vi "ContextManager.FGV.vi"(7 "context in":refnum<class "zmq_context.lvclass">, 10 "error in":errorcluster, 11 "action":T1) -> (2 "error out":errorcluster, 3 "context out":refnum<class "zmq_context.lvclass">, 5 "retired?":bool)   [LabVIEW 2019, in "RemoteControl.ZMQ.lvlib" / "ZMQ.ContextManager.lvlib"]
uses:
  ZMQ.ContextManager.lvlib
  <vilib>/addons/zeromq/zmq_context.lvclass
  Typedefs/Action--enum.ctl
  Typedefs/Context--Cluster.ctl
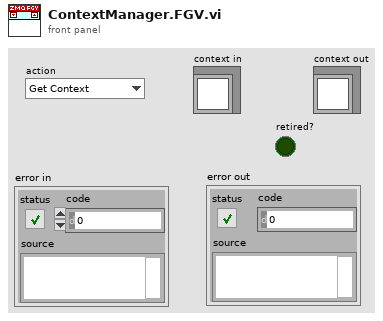
[diagram p1: front panel]
types:
  T1 = typedef "RemoteControl.ZMQ.lvlib/ZMQ.ContextManager.lvlib/Action--enum.ctl" = enum16{"Get Context", "Release Context", "Socket Opened", "Socket Closed", "Force Cleanup", "Set Context", "Retire If Idle"}
  T2 = typedef "RemoteControl.ZMQ.lvlib/ZMQ.ContextManager.lvlib/Context--Cluster.ctl" = cluster{"context":refnum<class "zmq_context.lvclass">, "context users":u32, "socket counter":u32, "idle since (ms)":u32}
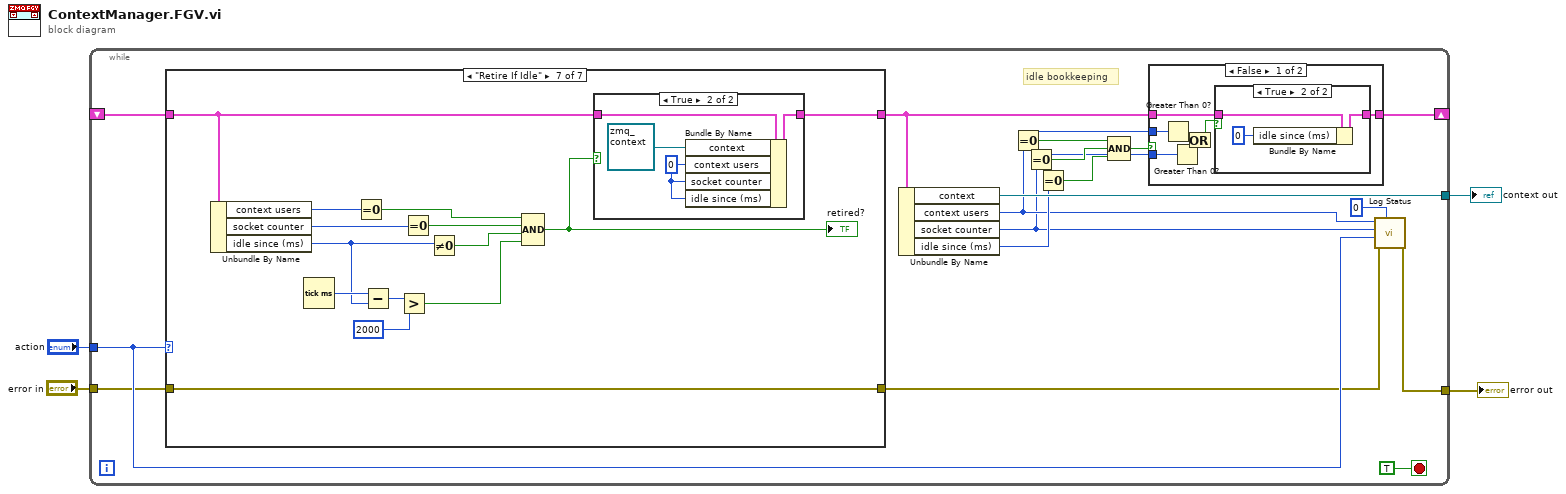
[diagram p0: block diagram]
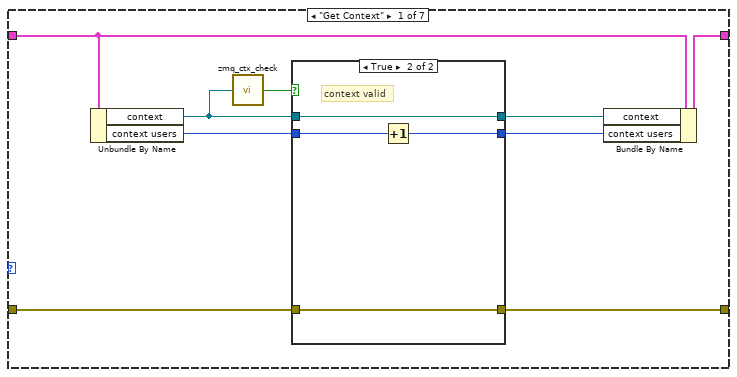
[diagram p2: hidden frame]
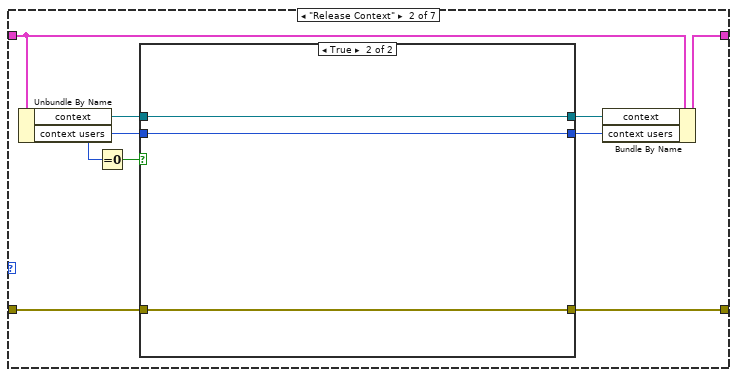
[diagram p4: hidden frame]
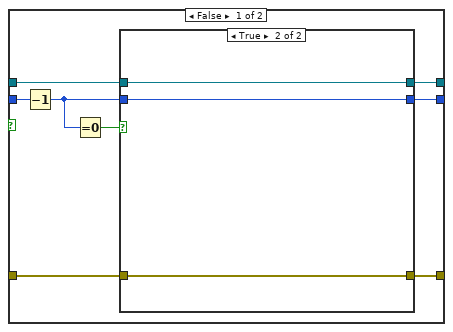
[diagram p5: hidden frame]
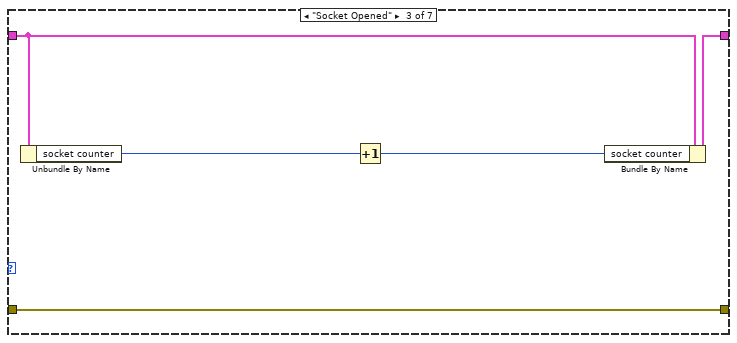
[diagram p7: hidden frame]
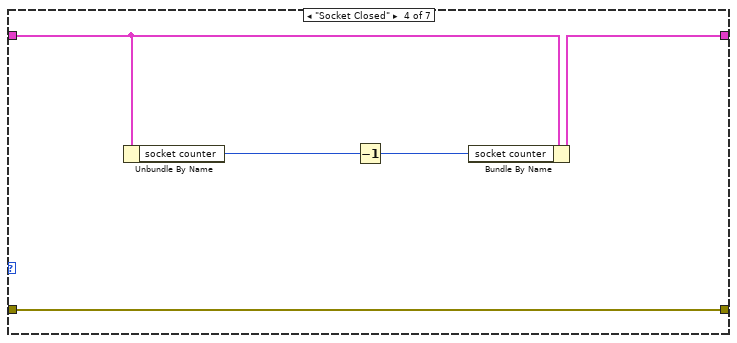
[diagram p8: hidden frame]
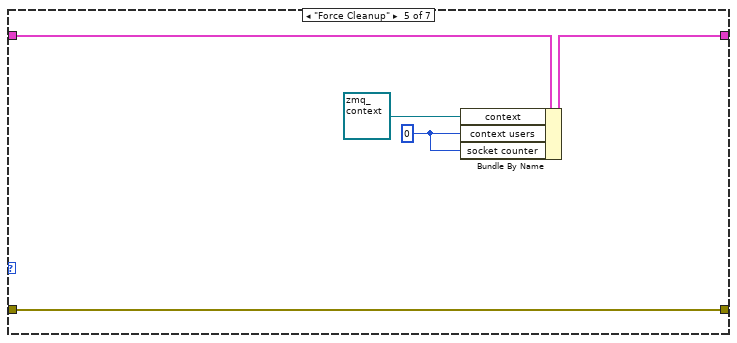
[diagram p9: hidden frame]
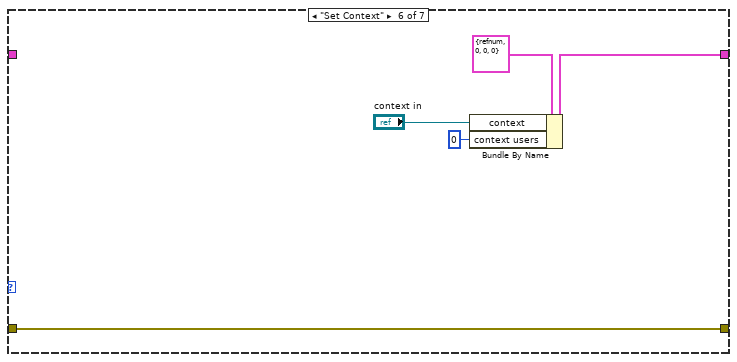
[diagram p10: hidden frame]
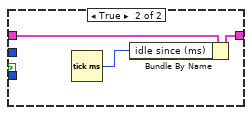
[diagram p13: hidden frame]
diagram:
  n1 = while {
    tunnel: "action" -> [w20]
    shift-right: [w11] -> _
    shift-left: _ -> [w16]
    tunnel: [w15] -> w3
    tunnel: "error in" -> [w19]
    tunnel: [w17] -> w1
    stop <- TRUE stop-if-true
    # "idle bookkeeping"
    n2 = case shown="\"Retire If Idle\"" w20 {
      tunnel: w19 -> [w30 w46 w68 w73 w74 w80 w95]
      tunnel: [w29 w45 w68 w73 w74 w80 w95] -> w18
      tunnel: w16 -> [w27 w42 w67 w72 w77 _ w90]
      tunnel: [w24 w41 w64 w69 w76 w83 w91] -> w13
      frame "Get Context" {
        n3 = Unbundle By Name(w27) -> ("context"=w28:refnum<class "zmq_context.lvclass">, "context users"=w23:u32)
        n4 = call <vilib>:"zmq_ctx_check.vi"("context in"=w28) -> ("valid?"=w22:bool)
        n5 = case shown="True" w22 {
          tunnel: [w33 w34] -> w26
          tunnel: w30 -> [w32 w37]
          tunnel: [w32 w37] -> w29
          tunnel: w23 -> [w31 w36]
          tunnel: [w31 w35] -> w25
          tunnel: w28 -> [w33 w34]
          frame False {
          }
          frame True {
            # "context valid"
            n6 = Increment(x=w36) -> (x+1=w35:u32)
          }
        }
        n7 = Bundle By Name(cluster=w27, "context"=w26, "context users"=w25) -> (w24:T2)
      }
      frame "Release Context" {
        n8 = Unbundle By Name(w42) -> ("context"=w40:refnum<class "zmq_context.lvclass">, "context users"=w38:u32)
        n9 = Equal To 0?(x=w38) -> (x = 0?=w39:bool)
        n10 = case shown="True" w39 {
          tunnel: w46 -> [w54 w61]
          tunnel: [w53 w61] -> w45
          tunnel: [w51 w62] -> w44
          tunnel: [w50 w63] -> w43
          tunnel: w40 -> [w49 w63]
          tunnel: w38 -> [w48 w62]
          frame False {
            n11 = Decrement(x=w48) -> (x-1=w47:u32)
            n12 = Equal To 0?(x=w47) -> (x = 0?=w52:bool)
            n13 = case shown="True" w52 {
              tunnel: w54 -> [w57 w60]
              tunnel: [w57 w60] -> w53
              tunnel: [w56 w58] -> w50
              tunnel: w49 -> [w56 w58]
              tunnel: [w55 w59] -> w51
              tunnel: w47 -> [w55 w59]
              frame False {
              }
              frame True {
              }
            }
          }
          frame True {
          }
        }
        n14 = Bundle By Name(cluster=w42, "context"=w43, "context users"=w44) -> (w41:T2)
      }
      frame "Socket Opened" {
        n15 = Unbundle By Name(w67) -> ("socket counter"=w66:u32)
        n16 = Increment(x=w66) -> (x+1=w65:u32)
        n17 = Bundle By Name(cluster=w67, "socket counter"=w65) -> (w64:T2)
      }
      frame "Socket Closed" {
        n18 = Unbundle By Name(w72) -> ("socket counter"=w71:u32)
        n19 = Decrement(x=w71) -> (x-1=w70:u32)
        n20 = Bundle By Name(cluster=w72, "socket counter"=w70) -> (w69:T2)
      }
      frame "Force Cleanup" {
        w75 = u32 0
        n21 = Bundle By Name(cluster=w77, "context"=refnum<class "zmq_context.lvclass"> refnum ("context out"), "context users"=w75, "socket counter"=w75) -> (w76:T2)
      }
      frame "Set Context" {
        n22 = Bundle By Name(cluster=T2 {"context"=refnum, "context users"=0, "socket counter"=0, "idle since (ms)"=0} ("data value"), "context"="context in", "context users"=u32 0) -> (w83:T2)
      }
      frame "Retire If Idle" {
        n23 = Unbundle By Name(w90) -> ("context users"=w96:u32, "socket counter"=w97:u32, "idle since (ms)"=w87:u32)
        n24 = Tick Count (ms)() -> (millisecond timer value=w88:u32)
        n25 = Equal To 0?(x=w96) -> (x = 0?=w94:bool)
        n26 = Subtract(x=w88, y=w87) -> (x-y=w86:u32)
        n27 = Greater?(x=w86, y=u32 2000) -> (0:w84:bool)
        n28 = Equal To 0?(x=w97) -> (x = 0?=w92:bool)
        n29 = Not Equal To 0?(x=w87) -> (x != 0?=w93:bool)
        n30 = Compound Arithmetic op=AND(w94, w92, w93, w84) -> (w89:bool)
        "retired?" <- w89
        n31 = case shown="True" w89 {
          tunnel: [w98 w102] -> w91
          tunnel: w90 -> [w98 w101]
          frame False {
          }
          frame True {
            w99 = u32 0 ("idle since (ms)")
            n32 = Bundle By Name(cluster=w101, "context"=refnum<class "zmq_context.lvclass"> refnum, "context users"=w99, "socket counter"=w99, "idle since (ms)"=w99) -> (w102:T2)
          }
        }
      }
    }
    n33 = Unbundle By Name(w13) -> ("context"=w15:refnum<class "zmq_context.lvclass">, "context users"=w6:u32, "socket counter"=w5:u32, "idle since (ms)"=w12:u32)
    n34 = Equal To 0?(x=w6) -> (x = 0?=w7:bool)
    n35 = Equal To 0?(x=w5) -> (x = 0?=w9:bool)
    n36 = Equal To 0?(x=w12) -> (x = 0?=w8:bool)
    n37 = Compound Arithmetic op=AND(w7, w9, w8) -> (w10:bool)
    n38 = case shown="False" w10 {
      tunnel: w13 -> [w108 w116]
      tunnel: [w109 w115] -> w11
      tunnel: w6 -> [w104 _]
      tunnel: w5 -> [w103 _]
      frame False {
        n39 = Greater Than 0?(x=w104) -> (x > 0?=w107:bool)
        n40 = Greater Than 0?(x=w103) -> (x > 0?=w106:bool)
        n41 = Or(x=w107, y=w106) -> (x .or. y?=w105:bool)
        n42 = case shown="True" w105 {
          tunnel: [w110 w113] -> w109
          tunnel: w108 -> [w110 w112]
          frame False {
          }
          frame True {
            n43 = Bundle By Name(cluster=w112, "idle since (ms)"=u32 0) -> (w113:T2)
          }
        }
      }
      frame True {
        n44 = Tick Count (ms)() -> (millisecond timer value=w114:u32)
        n45 = Bundle By Name(cluster=w116, "idle since (ms)"=w114) -> (w115:T2)
      }
    }
    n46 = call "Log Status.vi"("Context ID"=u32 0, "error in"=w18, "Action"=w20, "Socket Counter"=w5, "Context Counter"=w6) -> ("error out"=w17:errorcluster)  [unwired: 6 in]
  }
  "context out" <- w3
  "error out" <- w1
